vi "ACQ_SharedState_Transport_Auto.vi"() -> ()   [LabVIEW 2012]
panel:
  out "Queue cleanup error 2":errorcluster caption="sortie d'erreur"
  out "Queue cleanup error":errorcluster caption="sortie d'erreur"
  in  "packet":variant
  in  "Stop telemetry transport":bool
  out "Ack length in range (required)":bool
  out "Telemetry transport error only":errorcluster caption="sortie d'erreur"
  out "Ack JSON (raw; not validated)":string
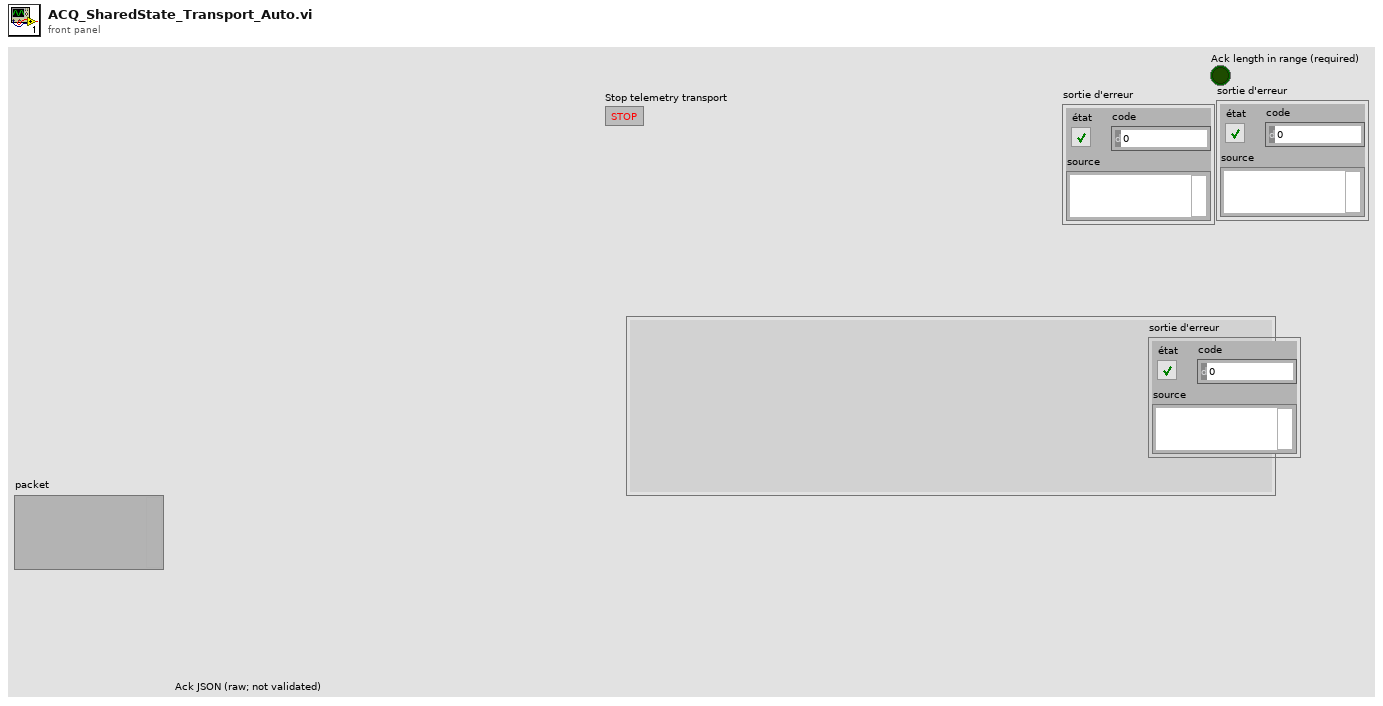
[diagram p1: front panel]
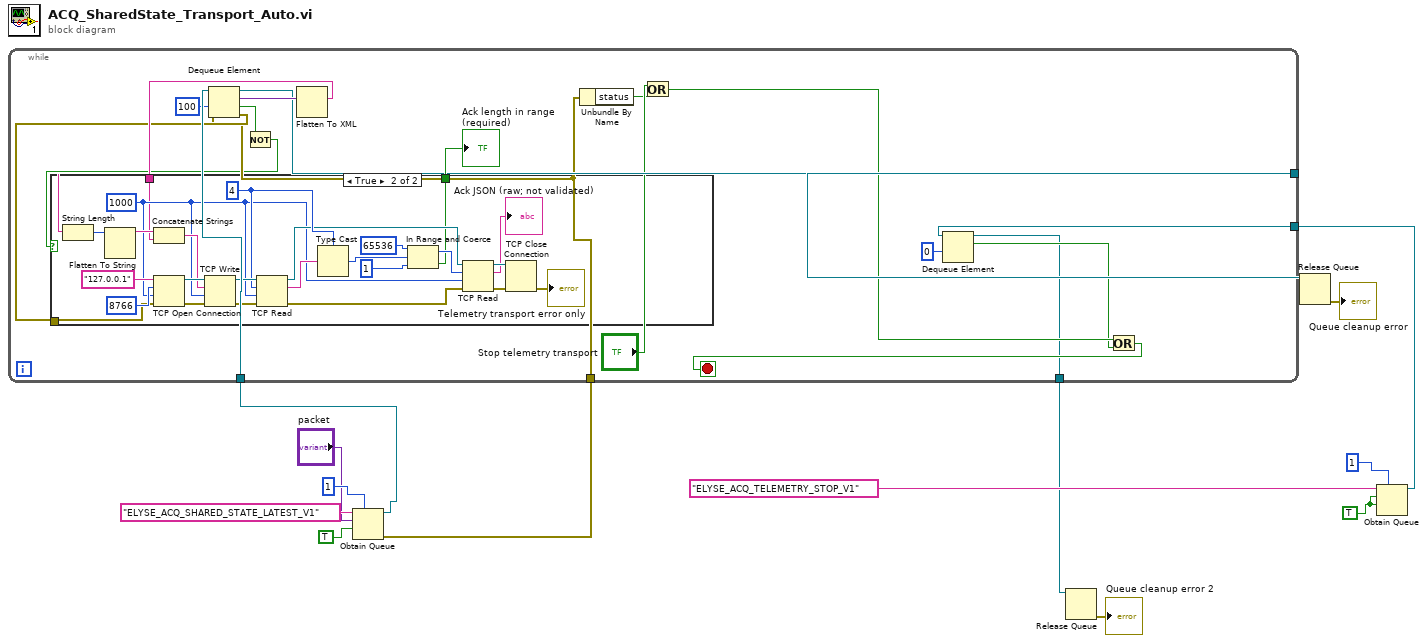
[diagram p0: block diagram]
diagram:
  w4 = TRUE ("créer si introuvable ? (V)")
  n1 = Obtain Queue(max queue size (-1, unlimited)=1 ("taille max de la file d'attente (-1, non limitée)"), name (unnamed)="ELYSE_ACQ_SHARED_STATE_LATEST_V1" ("nom (aucun)"), element data type="packet", create if not found? (T)=TRUE ("créer si introuvable ? (V)")) -> (queue out=w10:refnum<queue>, error out=w9:errorcluster)  [unwired: 1 in, 1 out]
  n2 = Obtain Queue(max queue size (-1, unlimited)=1 ("taille max de la file d'attente (-1, non limitée)"), name (unnamed)="ELYSE_ACQ_TELEMETRY_STOP_V1" ("nom (aucun)"), element data type=w4, create if not found? (T)=w4) -> (queue out=w3:refnum<queue>)  [unwired: 1 in, 2 out]
  n3 = while {
    tunnel: w10 -> [w31]
    tunnel: w9 -> [w25]
    tunnel: [w26] -> w8
    tunnel: w3 -> [w19]
    tunnel: [w15] -> w1
    stop <- w16 stop-if-true
    n4 = Dequeue Element(queue=w31, timeout in ms (-1)=100 ("timeout en ms (-1)"), error in (no error)=w25) -> (queue out=w26:refnum<queue>, element=w29:variant, timed out?=w22:bool, error out=w27:errorcluster)
    n5 = Not(x=w22) -> (.not. x?=w21:bool)
    n6 = Flatten To XML(anything=w29) -> (xml string=w28:string)
    n7 = case shown="True" w21 {
      tunnel: [_ w35] -> w32
      tunnel: w28 -> [_ w34]
      tunnel: w27 -> [_ w33]
      frame False {
      }
      frame True {
        w38 = 1000 ("timeout en ms (60000)")
        w48 = 4 ("octets à lire")
        n8 = String Length(string=w34) -> (length=w53:i32)
        n9 = Flatten To String(anything=w53) -> (data string=w52:string)  [unwired: 3 in, 2 out]
        n10 = Concatenate Strings(w52, w34) -> (w51:string)
        n11 = TCP Open Connection(address="127.0.0.1" ("adresse"), remote port or service name=u16 8766 ("port distant ou nom du service"), timeout ms (60000)=w38, error in (no error)=w33) -> (connection ID=w55:refnum<k5>, error out=w54:errorcluster)  [unwired: 1 in]
        n12 = TCP Write(connection ID=w55, data in=w51, error in (no error)=w54, 9:w38) -> (connection ID out=w50:refnum<k5>, error out=w49:errorcluster)  [unwired: 1 out]
        n13 = TCP Read(connection ID=w50, bytes to read=w48, error in (no error)=w49, 9:w38) -> (connection ID out=w46:refnum<k5>, data out=w47:string, error out=w45:errorcluster)  [unwired: 1 in]
        n14 = Type Cast(type=w48, x=w47) -> (*(type *) &x=w44:i32)
        n15 = In Range and Coerce(upper limit=65536 ("limite supérieure"), x=w44, lower limit=1 ("limite inférieure")) -> (coerced(x)=w41:i32, In Range?=w35:bool)
        n16 = TCP Read(connection ID=w46, bytes to read=w41, error in (no error)=w45, 9:w38) -> (connection ID out=w40:refnum<k5>, data out=→"Ack JSON (raw; not validated)":string, error out=w39:errorcluster)  [unwired: 1 in]
        n17 = TCP Close Connection(connection ID=w40, error in (no error)=w39) -> (error out=→"Telemetry transport error only":errorcluster)  [unwired: 1 in, 1 out]
      }
    }
    "Ack length in range (required)" <- w32
    n18 = Unbundle By Name(w25) -> ("status"=w23:bool)
    n19 = Or(x="Stop telemetry transport", y=w23) -> (x .or. y?=w18:bool)
    n20 = Dequeue Element(queue=w19, timeout in ms (-1)=0 ("timeout en ms (-1)")) -> (queue out=w15:refnum<queue>, element=w17:bool)  [unwired: 1 in, 2 out]
    n21 = Or(x=w18, y=w17) -> (x .or. y?=w16:bool)
  }
  n22 = Release Queue(queue=w1) -> (error out=→"Queue cleanup error 2":errorcluster)  [unwired: 2 in, 2 out]
  n23 = Release Queue(queue=w8) -> (error out=→"Queue cleanup error":errorcluster)  [unwired: 2 in, 2 out]
